vi "ZM-CM-evaluateError.vi"(8 "error in (no error)":errorcluster, 10 "stop actor? in":bool=TRUE, 11 "ZM-CM-communication_manager in":refnum<class "ZM-CM-communication_manager.lvclass">) -> (0 "error out":errorcluster, 2 "stop actor? out":bool=TRUE, 3 "ZM-CM-communication_manager out":refnum<class "ZM-CM-communication_manager.lvclass">)   [LabVIEW 2020, in "ZM-CM-communication_manager.lvlib" / "ZM-CM-communication_manager.lvclass"]
doc: "Error hook of the communication manager, called by Handle Error and after a helper loop. For now a pass-through: the class, the error and stop actor? go out unchanged; nothing is logged or cleared. Error-handling plan: none yet; an error stops the actor and, through its Last Ack, its caller."
uses:
  ZM-CM-communication_manager.lvclass
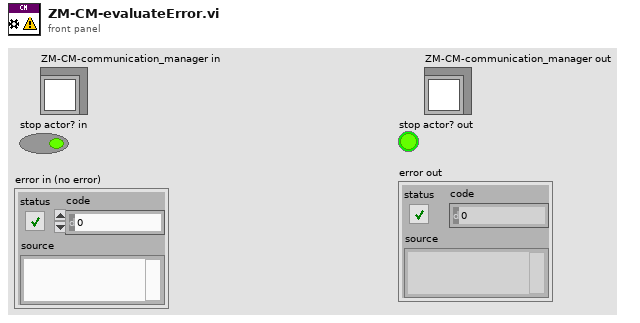
[diagram p1: front panel]
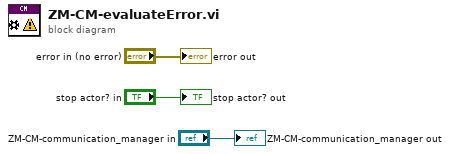
[diagram p0: block diagram]
diagram:
  "ZM-CM-communication_manager out" <- "ZM-CM-communication_manager in"
  "stop actor? out" <- "stop actor? in"
  "error out" <- "error in (no error)"
